vi "Set Log Folder.vi"(8 "error in (no error)":errorcluster, 10 "LogFolder":path, 11 "Node in":refnum<class "Node Config.lvclass">) -> (0 "error out":errorcluster, 3 "Node out":refnum<class "Node Config.lvclass">)   [LabVIEW 2020, in "VolatusConfig.lvlib" / "Node Config.lvclass"]
uses:
  Node Config.lvclass
  C:/dev/lv20CE/relink/lv-volatus/VolatusConfig/VolatusConfigElement/VolatusConfigElement.lvclass
  VolatusConfigElement/VolatusConfigElement.lvclass/VolatusConfigElement.ctl
  lv-cdm/CDM-Config/Path to String.vi
  lv-cdm/CDM-Config/Config Element/Write Variant Value.vi
  Node Config.lvclass/Node Config.ctl
  VolatusConfigElement/VolatusConfigElement.lvclass
  lv-cdm/CDM-Config/Config Element/Config Element.lvclass
  C:/dev/lv20CE/relink/lv-volatus/VolatusConfig/Node/Node Config.lvclass
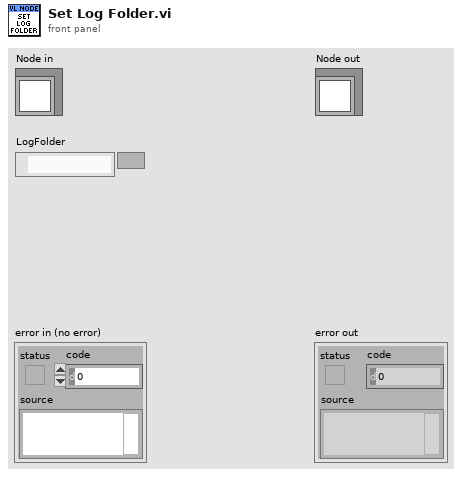
[diagram p1: front panel]
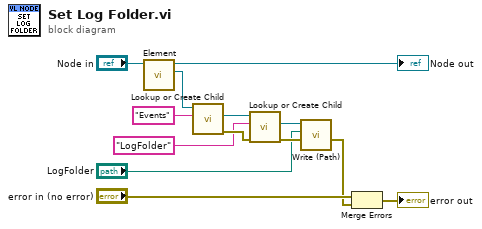
[diagram p0: block diagram]
diagram:
  n1 = call "Element.vi"("VolatusConfigElement in"="Node in") -> ("Element"=w10:refnum<class "Config Element.lvclass">, "VolatusConfigElement out"=→"Node out":refnum<class "Node Config.lvclass">)  [unwired: 9 in]
  n2 = call "Lookup or Create Child.vi"("Name"="Events", "Config Element in"=w10) -> ("error out"=w7:errorcluster, "Child"=w8:refnum<class "Config Element.lvclass">)  [unwired: 6 in, 2 out]
  n3 = call "Lookup or Create Child.vi"("error in (no error)"=w7, "Name"="LogFolder", "Config Element in"=w8) -> ("error out"=w5:errorcluster, "Child"=w4:refnum<class "Config Element.lvclass">)  [unwired: 5 in, 2 out]
  n4 = call "Write (Path).vi"("error in (no error)"=w5, "Path Value"="LogFolder", "Config Element in"=w4) -> ("error out"=w1:errorcluster)  [unwired: 7 in, 1 out]
  n5 = Merge Errors("error in (no error)", w1) -> (→"error out":errorcluster)
